vi "Read configuration.vi"(8 "error in (no error)":errorcluster, 11 "PAC Channel in":refnum<class "PAC Channel.lvclass">) -> (0 "error out":errorcluster, 2 "configuration":refnum<class "CEF_serializable configuration.lvclass">, 3 "PAC Channel out":refnum<class "PAC Channel.lvclass">)   [LabVIEW 2025, in "PAC.lvlib" / "PAC Channel.lvclass"]
uses:
  PAC Channel.lvclass
  PAC Channel.lvclass/PAC Channel.ctl
  PAC Channel configuration/PAC Channel configuration.lvclass
  Users/Public/Documents/Sandia National Labs/TSS Plugin/CEF.lvlibp/serializable configuration/CEF_serializable configuration.lvclass
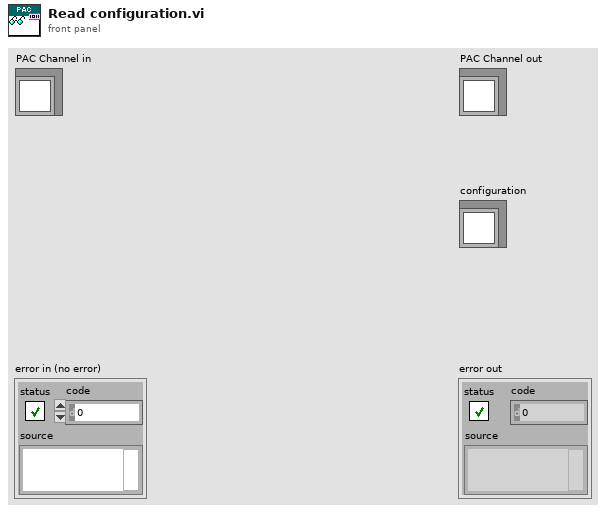
[diagram p1: front panel]
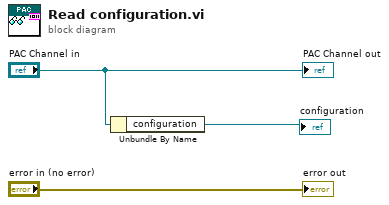
[diagram p0: block diagram]
diagram:
  n1 = Unbundle By Name("PAC Channel in") -> ("configuration"=→"configuration":refnum<class "PAC Channel configuration.lvclass">)
  "error out" <- "error in (no error)"
  "PAC Channel out" <- "PAC Channel in"
